vi "Orca Flash Data Spooler.vi"(7 "Calling VI Ref":refnum<vi>) -> ()   [LabVIEW 2016]
uses:
  <vilib>/vision/Image Controls.llb/IMAQ Image.ctl
  Orca Flash Capture Manager Controls/Orca Flash Capture Notifier Type.ctl
  Orca Flash Capture Manager Controls/Orca Flash Capture Actions.ctl
  Orca Flash Capture Manager Controls/Orca Flash Capture Switch Line Scan Modes.ctl
  Orca Flash Data Spooler/Orca Data Spooler Type Defs/Orca Data Spooler Notifier Type.ctl
  Orca Flash Data Spooler/Orca Data Spooler Type Defs/Orca Data Spooler Actions.ctl
  <vilib>/Utility/miscctls.llb/LVPointTypeDef.ctl
  Orca Flash Data Spooler/Orca Data Spooler Type Defs/Orca Data Spooler Transfer Data.ctl
  Orca Flash Data Spooler/Orca Data Spooler Type Defs/Orca Data Spooler Last Used.ctl
  Orca Flash Data Spooler/Orca Data Spooler Type Defs/Orca Data Spooler Transfer Log Type.ctl
  Tools/Copy File with Progress/Copy File DLL/x64/Release/Copy File DLL.dll
panel:
  in  "Main Tab":enum32{"Data Spooler", "Remote Queue"}(tab)
  out "Source Path":string
  out "Destination Path":string
  in  "Set Destination":bool
  in  "Disable Spooler":bool
  in  "Auto Match Paths":bool=TRUE
  in  "Skip File":bool
  in  "Abort":bool
  out "Copy Success":bool
  out "Current File":string
  out "Transfer Amount (%)":u8
  out "Spooler Active":bool
  out "Queue Started":bool
  in  "Open Queue":bool
  in  "Quit":bool
  out "Start Up Error":errorcluster
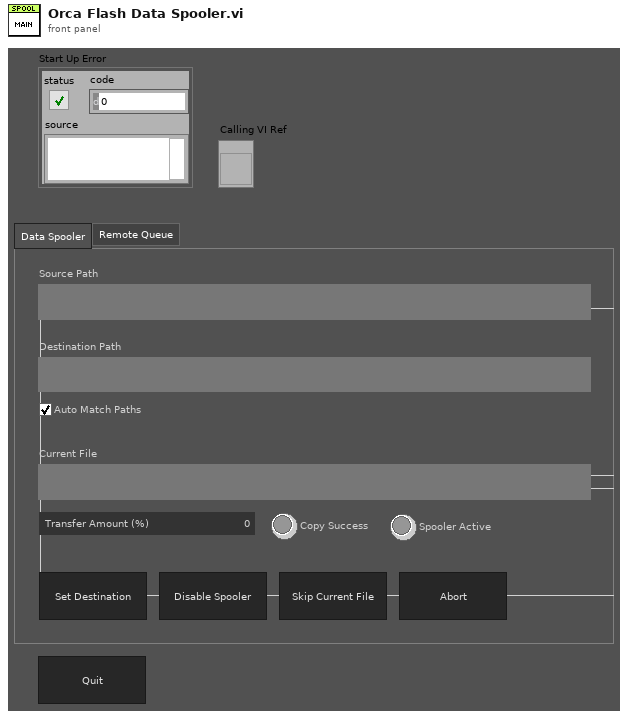
[diagram p1: front panel]
types:
  T1 = typedef "Orca Data Spooler Transfer Data.ctl" = cluster{"transLogPath":string, "imageName":string, "noFrames":u32, "noCycles":u16, "quitFlag":bool, "channelCode":u8, "setupName":string}
  T2 = enum16{"Always On", "Always Off", "Off While Running"}
  T3 = typedef "LVPointTypeDef.ctl" = cluster{"Horizontal":i16, "Vertical":i16}
  T4 = typedef "Orca Data Spooler Actions.ctl" = enum16{"Idle", "Start Spooler", "Update Destination", "Create Log File", "Wait for File", "Update Log", "Copy File", "Copy JSON Files", "Log Done", "Abort", "Exit", "Quit"}
  T5 = typedef "Orca Data Spooler Notifier Type.ctl" = cluster{"Actions":T4, "Source":path, "Destination":path, "Running?":bool, "Transfer Log":path}
  T6 = enum8{"Enabled", "Disabled", "Disabled and Grayed Out"}
  T7 = typedef "Orca Flash Capture Notifier Type.ctl" = cluster{"Actions":T8, "Running?":bool, "Preview Exposure (s)":dbl, "Capture Exposure (s)":dbl, "Cycles":u16, "Frames":u32, "No. of Z Steps":u16, "Z Step Size (µm)":dbl, "Base Path":path, "Init Z Position (µm)":dbl, "Lasers Lines":string[], "Save Path":path, "Line Scan?":bool, "Line Scan Mode":T9, "Collect Metadata?":bool, "channelCode":u8, "setupName":string}
  T8 = typedef "Orca Flash Capture Actions.ctl" = enum16{"Idle", "Live Preview", "Capture", "Check File Name", "Laser On", "Laser Off", "Open Shutters", "Close Shutters", "Set Exposure Time", "Start Acquisition", "Update SubFolder", "Write Metadata", "Setup", "Camera", "Switch", "Step", "Cycle", "External Cycle Sync", "Abort", "Quit"}
  T9 = typedef "Orca Flash Capture Switch Line Scan Modes.ctl" = enum32{"Automatic", "Use Presets", "Manual"}
  T10 = typedef "IMAQ Image.ctl" = refnum<image>
  T11 = cluster{"Image Ref":T10, "Cycle Number":u16, "Camera Running?":bool, "Capture?":bool}
  T12 = enum32{"Bad", "Idle", "Run top level", "Running"}
  T13 = typedef "Orca Data Spooler Last Used.ctl" = cluster{"Source":string, "Destination":string}
  T14 = typedef "LVRectTypeDef.ctl" = cluster{"Left":i16, "Top":i16, "Right":i16, "Bottom":i16}
  T15 = typedef "LVBoundsTypeDef.ctl" = cluster{"Width":u32, "Height":u32}
  T16 = enum16{"open", "replace", "create", "open or create", "replace or create", "replace or create with confirmation"}
  T17 = typedef "Orca Data Spooler Transfer Log Type.ctl" = cluster{"File Name":string, "Status":string}
  T18 = enum32{"Invalid", "Standard", "Closed", "Hidden", "Minimized", "Maximized"}
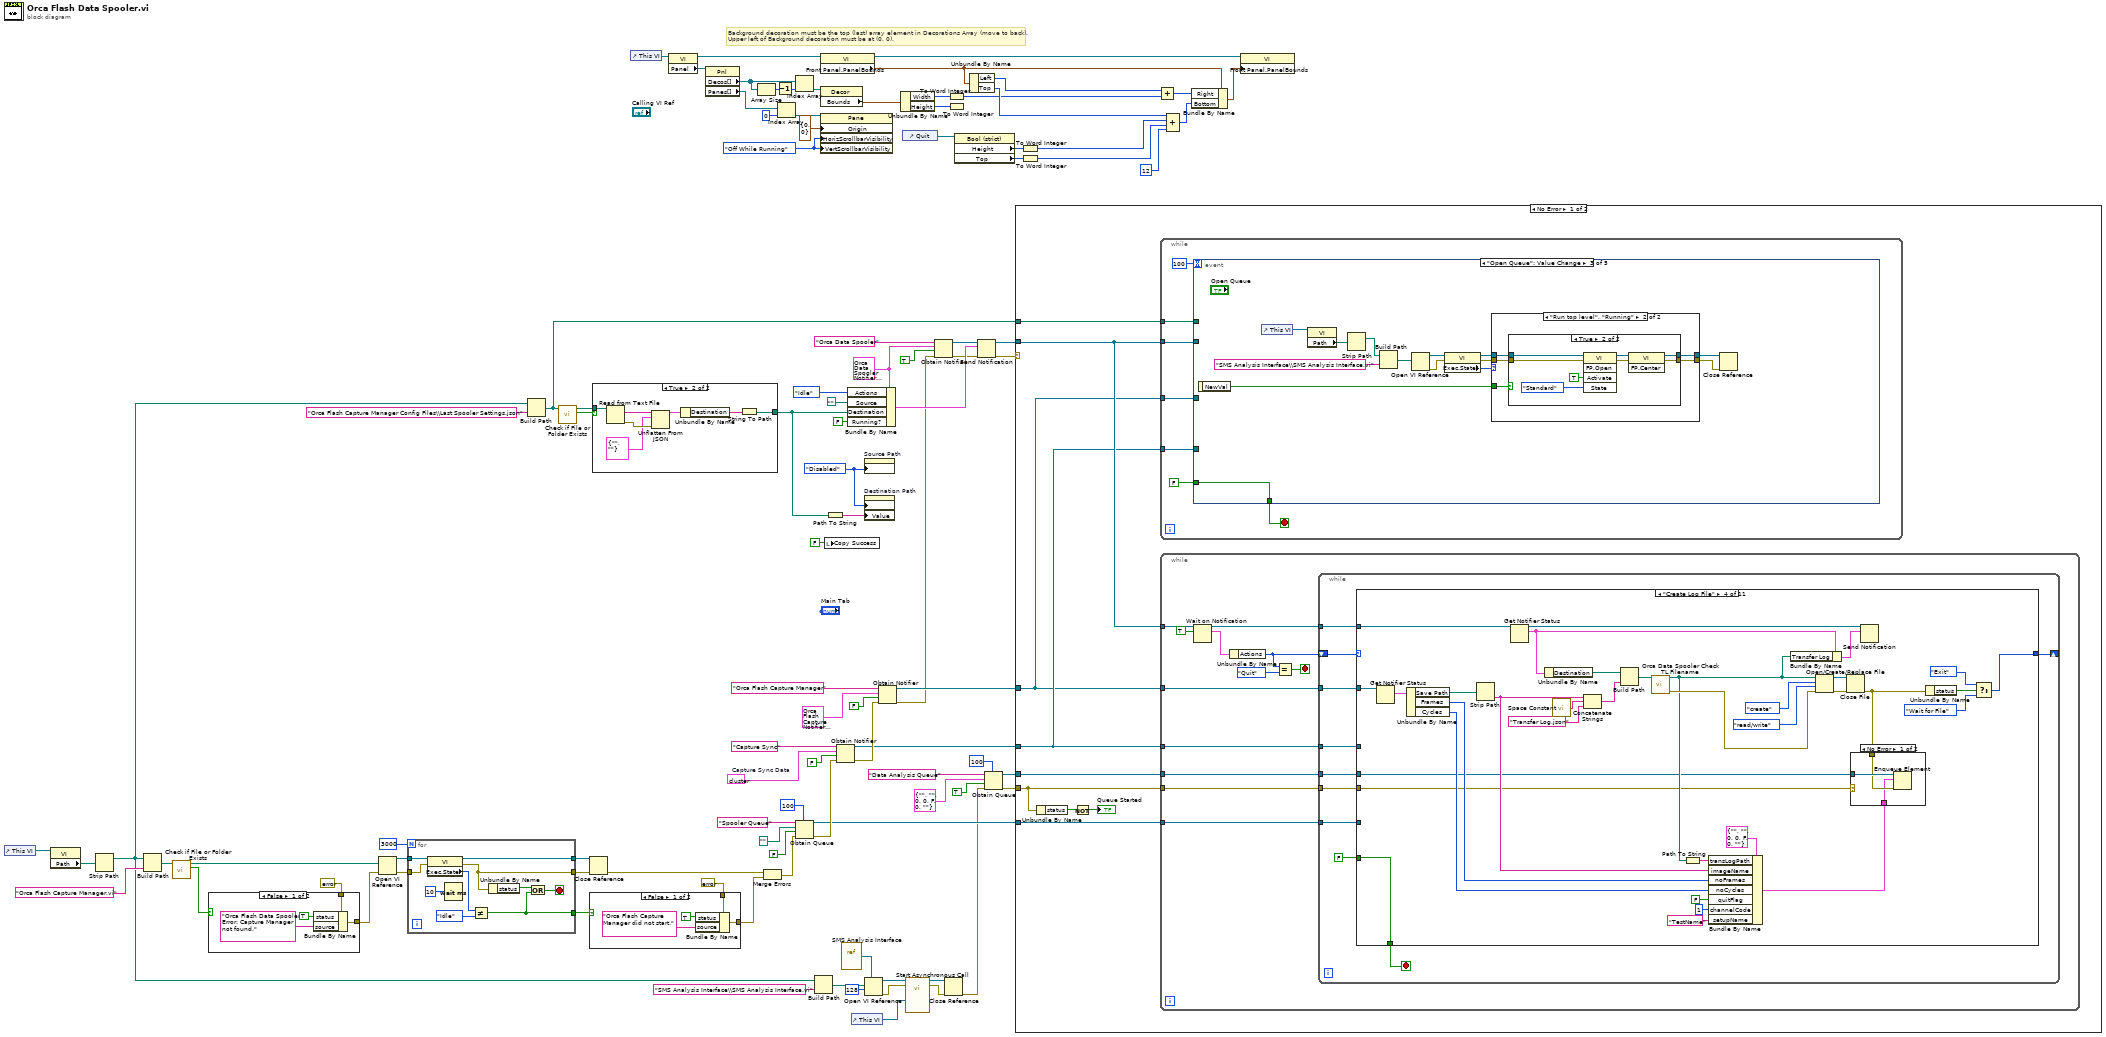
[diagram p0: block diagram]
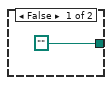
[diagram p2: hidden frame]
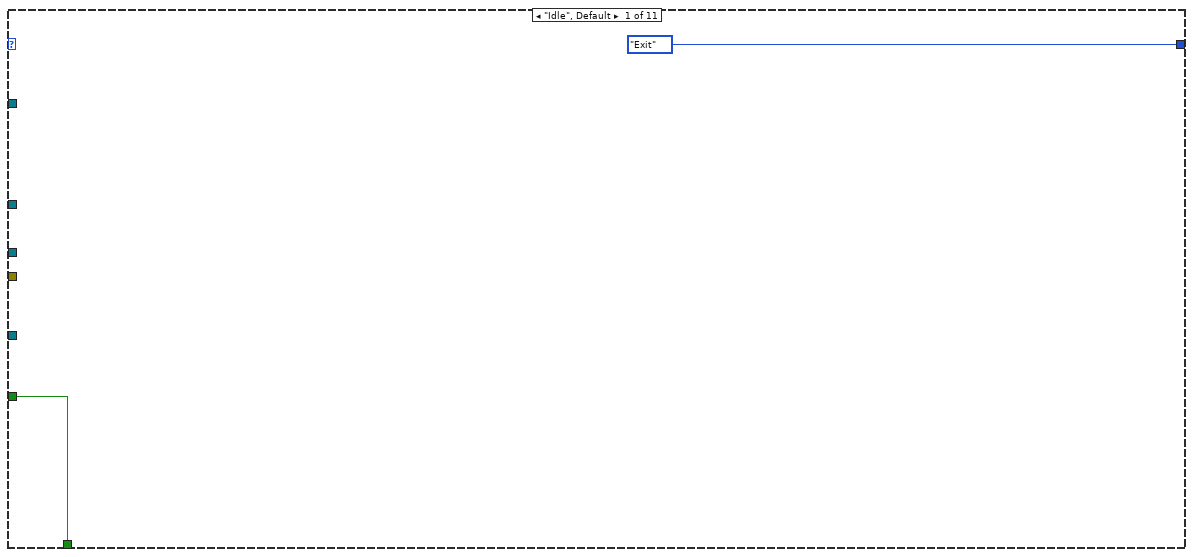
[diagram p3: hidden frame]
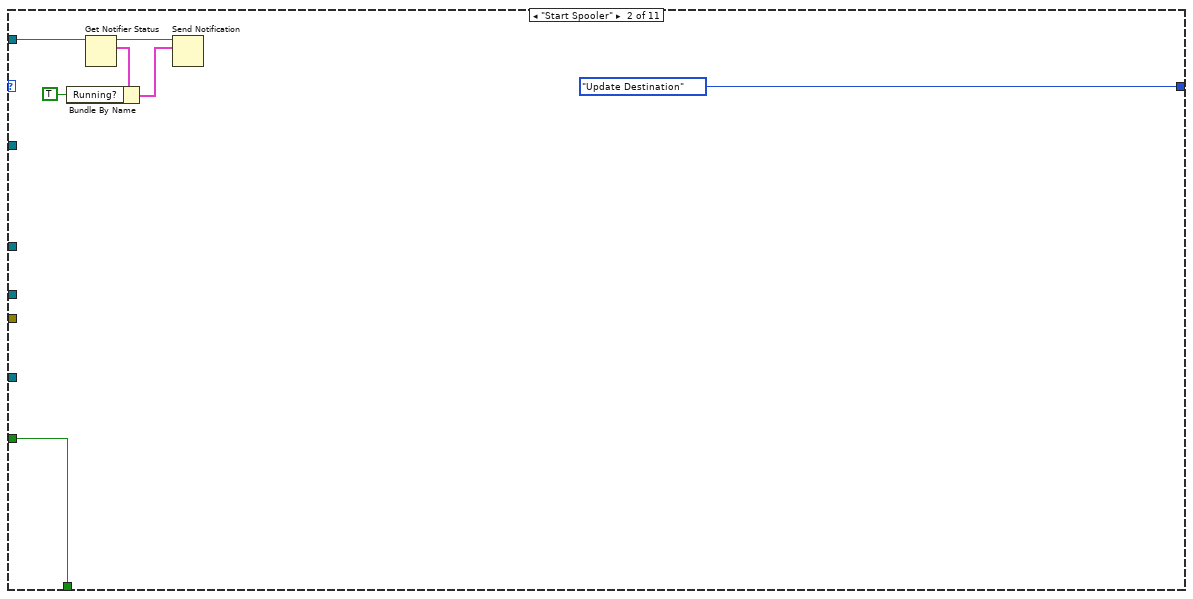
[diagram p4: hidden frame]
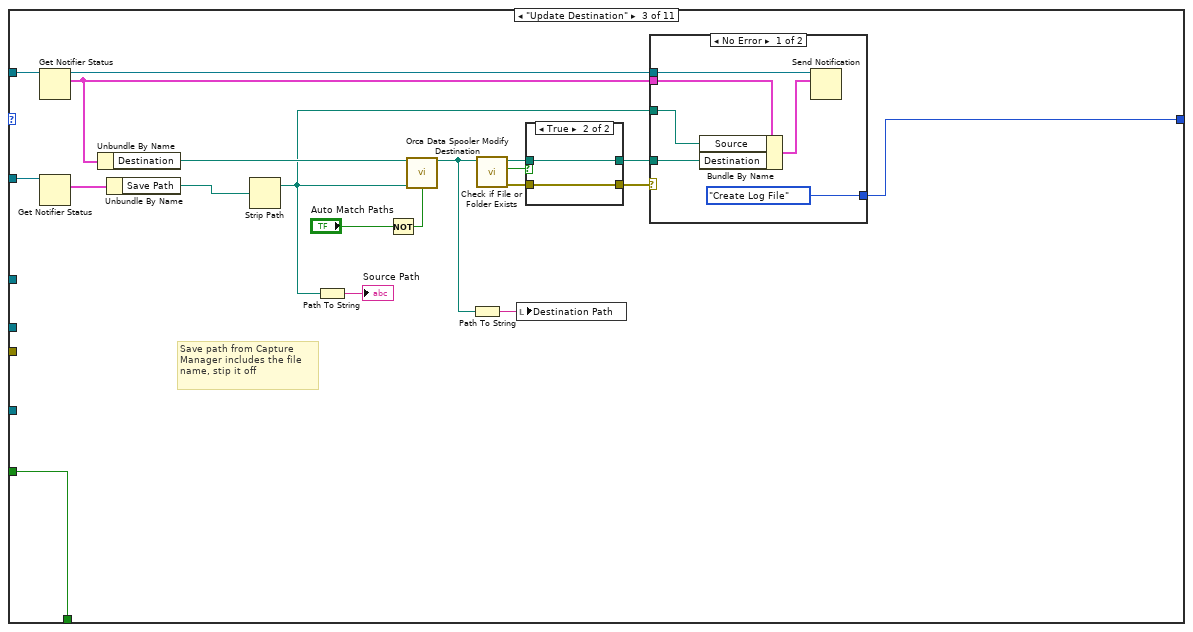
[diagram p5: hidden frame]
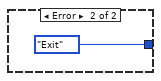
[diagram p6: hidden frame]
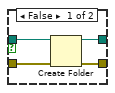
[diagram p7: hidden frame]
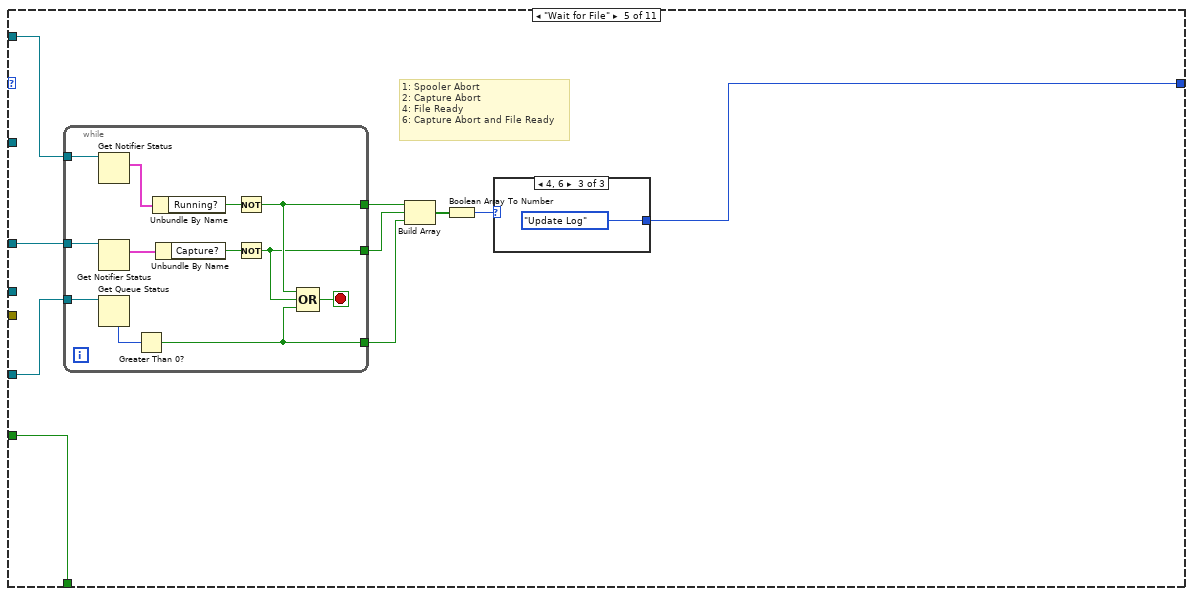
[diagram p9: hidden frame]
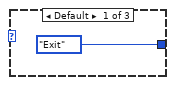
[diagram p10: hidden frame]
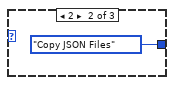
[diagram p11: hidden frame]
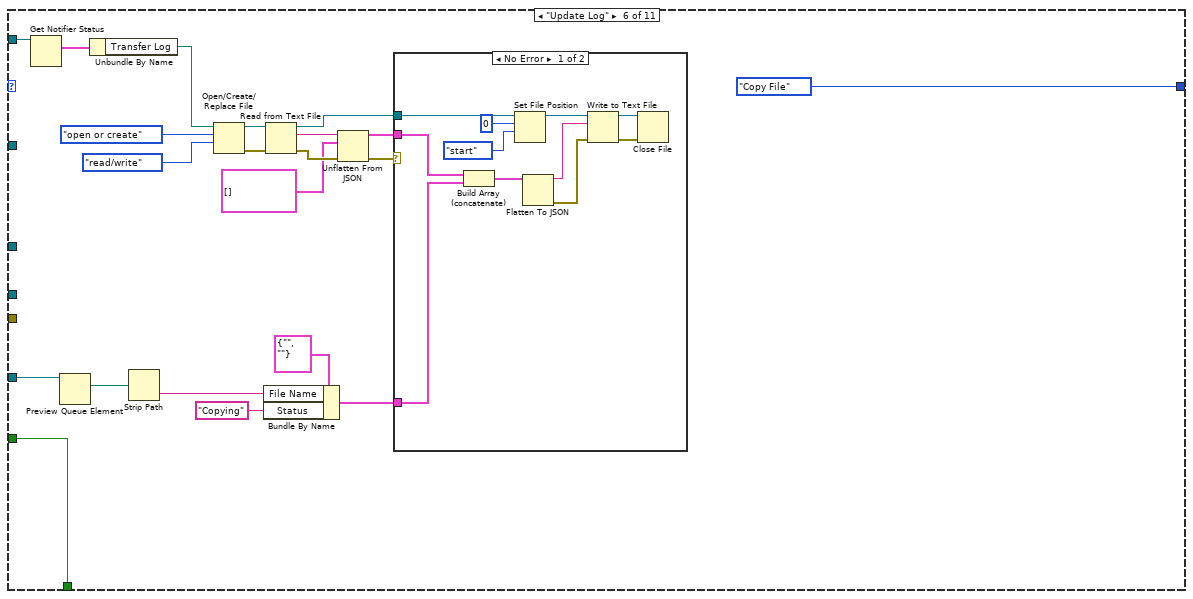
[diagram p12: hidden frame]
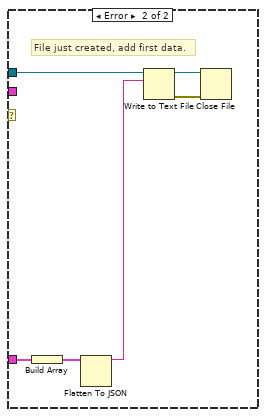
[diagram p13: hidden frame]
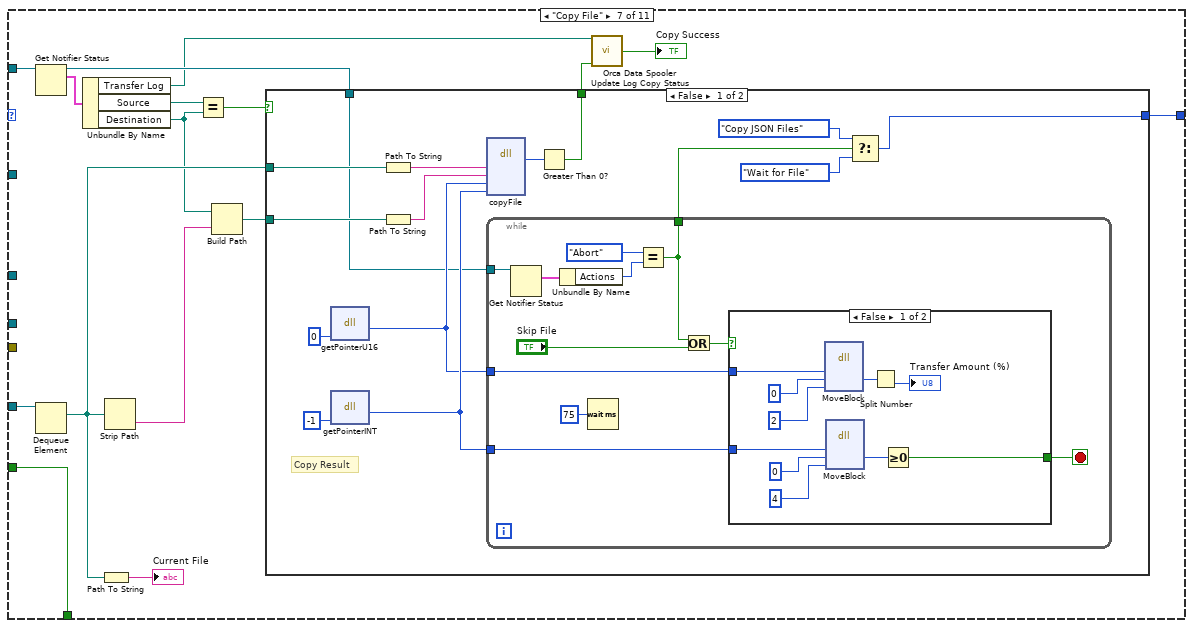
[diagram p14: hidden frame]
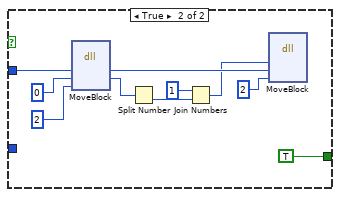
[diagram p15: hidden frame]
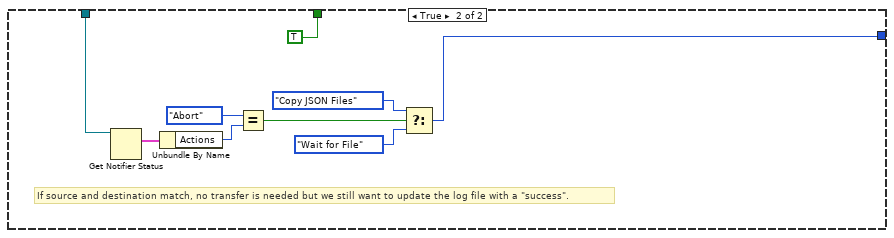
[diagram p16: hidden frame]
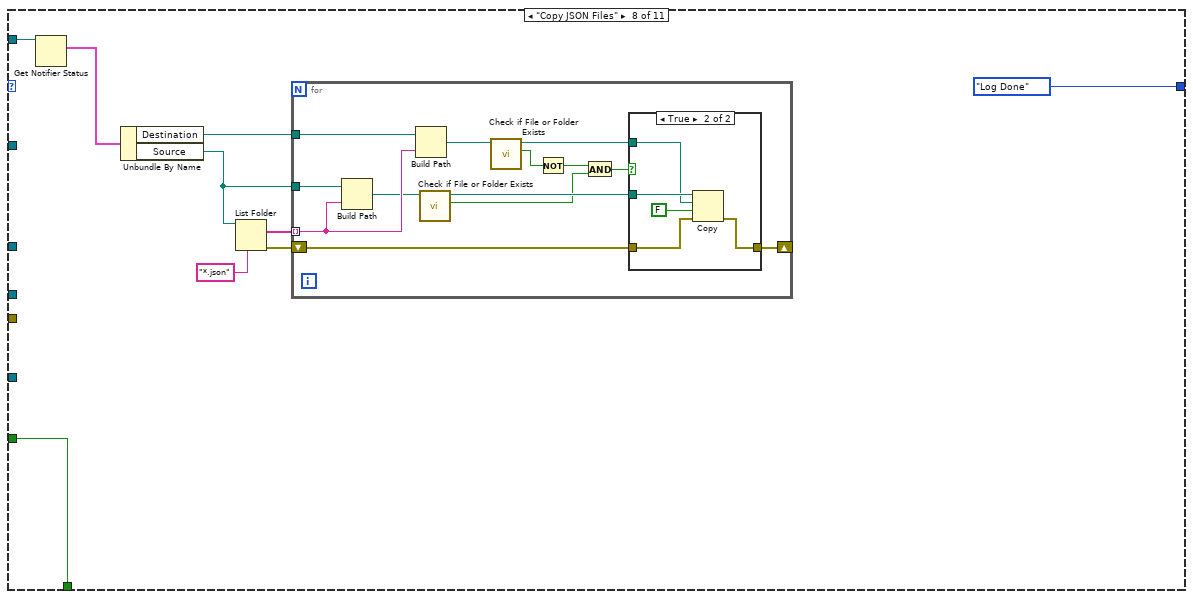
[diagram p17: hidden frame]
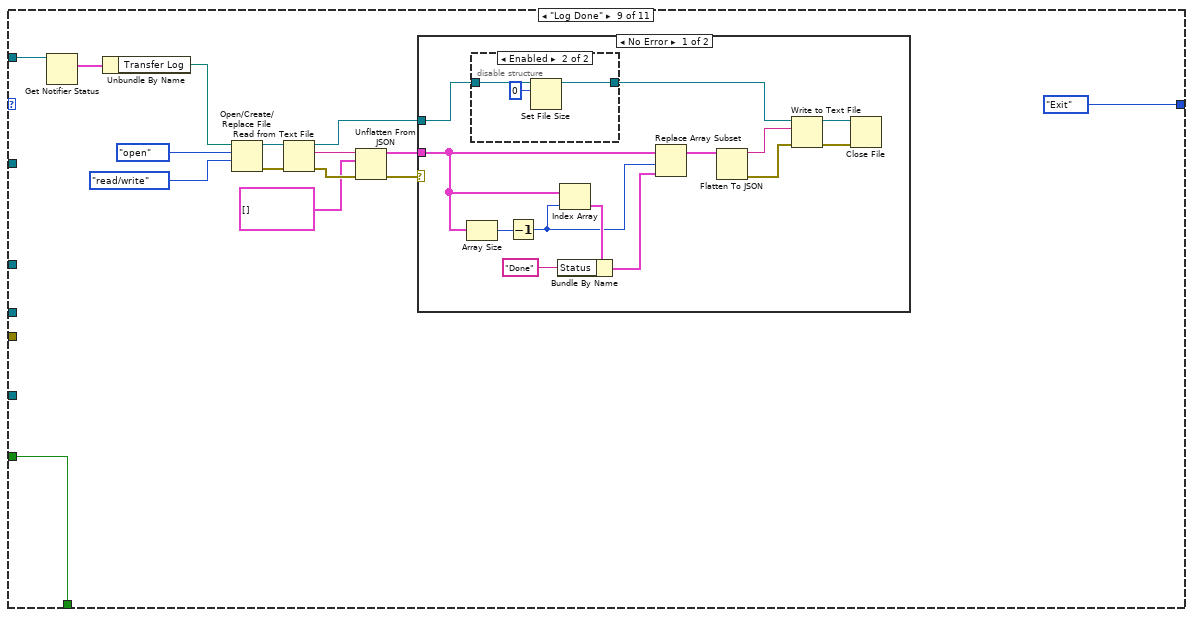
[diagram p19: hidden frame]
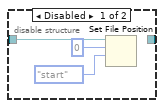
[diagram p20: hidden frame]
diagram:
  w39 = T2."Off While Running" ("Vertical Scrollbar Visibility")
  w65 = T5 {"Actions"=enum."Idle", "Source"=path "", "Destination"=path "", "Running?"=FALSE, "Transfer Log"=path ""} ("Orca Data Spooler Notifier Type")
  w71 = T6."Disabled" ("Disabled")
  w86 = T11 {"Image Ref"=refnum, "Cycle Number"=0, "Camera Running?"=FALSE, "Capture?"=FALSE}  # Capture Sync Data
  # "Background decoration must be the top (last) array element in Decorations Array (move to back).\nUpper left of Background decoration must be at (0, 0)."
  n1 = control-ref of="This VI"() -> (w99:refnum<vi>)
  n2 = property class="VI"(reference=w99) -> ("Path"=w98:path)  [unwired: 1 in, 2 out]
  n3 = Strip Path(path=w98) -> (stripped path=w10:path)  [unwired: 1 out]
  n4 = Build Path(base path=w10, name or relative path="Orca Flash Capture Manager.vi" ("name (unnamed)")) -> (appended path=w96:path)
  n5 = call <vilib>:"Check if File or Folder Exists.vi"("path"=w96) -> ("file or folder exists?"=w95:bool, "dup path"=w92:path)  [unwired: 8 in, 1 out]
  n6 = case shown="False" w95 {
    tunnel: errorcluster {"status"=FALSE, "code"=0, "source"=""} ("error in (no error)") -> [w101 w104]
    tunnel: [w100 w104] -> w91
    frame False {
      n7 = Bundle By Name(cluster=w101, "status"=TRUE, "source"="Orca Flash Data Spooler Error: Capture Manager not found." ("name (unnamed)")) -> (w100:errorcluster)
    }
    frame True {
    }
  }
  n8 = Open VI Reference(vi path=w92, error in (no error)=w91) -> (vi reference=w93:refnum<vi>, error out=w87:errorcluster)  [unwired: 4 in]
  n9 = for {
    N: 3000 -> [_]
    tunnel: w93 -> [w114]
    tunnel: [w110] -> w89
    tunnel: [w105] -> w79
    tunnel: [w107] -> w88
    tunnel: w87 -> [w106]
    stop <- w108 stop-if-true
    n10 = property class="VI"(reference=w114, error in=w106) -> (reference out=w110:refnum<vi>, error out=w107:errorcluster, "Exec.State"=w112:T12)
    n11 = Wait (ms)(milliseconds to wait=u32 10) -> ()  [unwired: 1 out]
    n12 = Not Equal?(x=w112, y=T12."Idle") -> (x != y?=w105:bool)
    n13 = Unbundle By Name(w107) -> ("status"=w109:bool)
    n14 = Or(x=w109, y=w105) -> (x .or. y?=w108:bool)
  }
  n15 = Build Path(base path=w10, name or relative path="Orca Flash Capture Manager Config Files\\Last Spooler Settings.json" ("name (unnamed)")) -> (appended path=w19:path)
  n16 = call <vilib>:"Check if File or Folder Exists.vi"("path"=w19) -> ("file or folder exists?"=w68:bool, "dup path"=w69:path)  [unwired: 8 in, 1 out]
  n17 = Close Reference(reference=w89, error in (no error)=w88) -> (error out=w78:errorcluster)
  n18 = case shown="False" w79 {
    tunnel: errorcluster {"status"=FALSE, "code"=0, "source"=""} ("error in (no error)") -> [w116 w119]
    tunnel: [w115 w119] -> w77
    frame False {
      n19 = Bundle By Name(cluster=w116, "status"=TRUE, "source"="Orca Flash Capture Manager did not start." ("name (unnamed)")) -> (w115:errorcluster)
    }
    frame True {
    }
  }
  n20 = case shown="True" w68 {
    tunnel: w69 -> [_ w125]
    tunnel: [path "" w121] -> w61
    frame False {
    }
    frame True {
      n21 = Read from Text File(file (use dialog)=w125) -> (text=w127:string, error out=w126:errorcluster)  [unwired: 3 in, 2 out]
      n22 = Unflatten From JSON(JSON string=w127, type and defaults=T13 {"Source"="", "Destination"=""} ("Orca Data Spooler Notifier Type"), error in (no error)=w126) -> (value=w123:T13)  [unwired: 4 in, 1 out]
      n23 = Unbundle By Name(w123) -> ("Destination"=w122:string)
      n24 = String To Path(string=w122) -> (path=w121:path)
    }
  }
  n25 = control-ref of="This VI"() -> (w31:refnum<vi>)
  n26 = property class="VI"(reference=w31) -> (reference out=w40:refnum<vi>, "Panel"=w32:refnum<vi>)  [unwired: 1 in, 1 out]
  n27 = property class="Pnl"(reference=w32) -> ("Decos[]"=w30:refnum<vi>[], "Panes[]"=w36:refnum<vi>[])  [unwired: 1 in, 2 out]
  n28 = Array Size(array=w30) -> (size(s)=w28:i32)
  n29 = Merge Errors(w78, w77) -> (w22:errorcluster)
  n30 = Decrement(x=w28) -> (x-1=w29:i32)
  n31 = Index Array(array=w36, index=0) -> (element=w35:refnum<vi>)
  n32 = Index Array(array=w30, index=w29) -> (element=w38:refnum<vi>)
  n33 = Obtain Queue(max queue size (-1, unlimited)=100, name (unnamed)="Spooler Queue", element data type=path "", create if not found? (T)=FALSE, error in (no error)=w22) -> (queue out=w20:refnum<queue>, error out=w21:errorcluster)  [unwired: 1 out]
  n34 = Build Path(base path=w10, name or relative path="SMS Analysis Interface\\SMS Analysis Interface.vi" ("name (unnamed)")) -> (appended path=w11:path)
  n35 = property class="VI"(reference=w40) -> (reference out=w42:refnum<vi>, "Front Panel.PanelBounds"=w43:T14)  [unwired: 1 in, 1 out]
  n36 = property class="Decor"(reference=w38) -> ("Bounds"=w41:T15)  [unwired: 1 in, 2 out]
  n37 = property class="Pane"(reference=w35, "Origin"=T3 {"Horizontal"=0, "Vertical"=0}, "HorizScrollbarVisibility"=w39, "VertScrollbarVisibility"=w39) -> ()  [unwired: 1 in, 2 out]
  n38 = local write "Copy Success"(FALSE ("Copy Success")) -> ()
  n39 = Path To String(path=w61) -> (string=w60:string)
  n40 = Obtain Notifier(name (unnamed)="Capture Sync", notification data type=w86, create if not found? (T)=FALSE, error in (no error)=w21) -> (notifier out=w74:refnum<notifier>, error out=w76:errorcluster)  [unwired: 1 out]
  n41 = vi-ref "SMS Analysis Interface.vi"() -> (w9:refnum<vi>)
  n42 = Bundle By Name(cluster=w65, "Actions"=Orca_Data_Spooler_Actions."Idle", "Source"=path "", "Destination"=w61, "Running?"=FALSE) -> (w63:T5)
  n43 = control-ref of="This VI"() -> (w3:refnum<vi>)
  n44 = property on="Source Path" class="Str"("DisabledEnum"=w71) -> ()  [unwired: 2 in, 2 out]
  n45 = property on="Destination Path" class="Str"("DisabledEnum"=w71, "Value"=w60) -> ()  [unwired: 2 in, 2 out]
  n46 = Open VI Reference(type specifier VI Refnum (for type only)=w9, vi path=w11, options=128) -> (vi reference=w7:refnum<vi>, error out=w5:errorcluster)  [unwired: 3 in]
  n47 = Obtain Notifier(name (unnamed)="Orca Flash Capture Manager", notification data type=T7 {"Actions"=enum."Live Preview", "Running?"=FALSE, "Preview Exposure (s)"=0.1, "Capture Exposure (s)"=0.1, "Cycles"=1, "Frames"=0, "No. of Z Steps"=0, "Z Step Size (µm)"=0.0, "Base Path"=path "", "Init Z Position (µm)"=0.0, "Lasers Lines"=[], "Save Path"=path "", "Line Scan?"=FALSE, "Line Scan Mode"=enum."Automatic", "Collect Metadata?"=FALSE, "channelCode"=0, "setupName"=""} ("4Pi Capture Notifier Type"), create if not found? (T)=FALSE, error in (no error)=w76) -> (notifier out=w75:refnum<notifier>, error out=w59:errorcluster)  [unwired: 1 out]
  n48 = Unbundle By Name(w41) -> ("Width"=w46:u32, "Height"=w49:u32)
  n49 = control-ref of="Quit"() -> (w33:refnum<vi>)
  n50 = call-by-ref "Start Asynchronous Call"(reference=w7, error in=w5, "Calling VI Ref"=w3) -> (reference out=w6:refnum<vi>, error out=w4:errorcluster)  [unwired: 15 in]
  n51 = Obtain Notifier(name (unnamed)="Orca Data Spooler", notification data type=w65, create if not found? (T)=TRUE, error in (no error)=w59) -> (notifier out=w64:refnum<notifier>, error out=w62:errorcluster)  [unwired: 1 out]
  n52 = Close Reference(reference=w6, error in (no error)=w4) -> (error out=w2:errorcluster)
  n53 = To Word Integer(number=w46) -> (16bit integer=w48:i16)
  n54 = To Word Integer(number=w49) -> ()  [unwired: 1 out]
  n55 = property class="Bool (strict)"(reference=w33) -> ("Height"=w51:u32, "Top"=w52:i32)  [unwired: 1 in, 2 out]
  n56 = Unbundle By Name(w43) -> ("Left"=w45:i16, "Top"=w56:i16)
  n57 = Send Notification(notification=w63, notifier=w64, error in (no error)=w62) -> (notifier out=w57:refnum<notifier>, error out=w58:errorcluster)
  n58 = Obtain Queue(max queue size (-1, unlimited)=100, name (unnamed)="Data Analysis Queue", element data type=T1 {"transLogPath"="", "imageName"="", "noFrames"=0, "noCycles"=0, "quitFlag"=FALSE, "channelCode"=0, "setupName"=""} ("Spooler Connection Data"), create if not found? (T)=TRUE, error in (no error)=w2) -> (queue out=w13:refnum<queue>, error out=w1:errorcluster)  [unwired: 1 out]
  n59 = case shown="No Error" w58 {
    selector: w58 -> [_ w552]
    tunnel: w75 -> [w134 w550]
    tunnel: w74 -> [w135 w548]
    tunnel: w57 -> [w136 w549]
    tunnel: w20 -> [w133 _]
    tunnel: w19 -> [w132 _]
    tunnel: w13 -> [w131 _]
    tunnel: w1 -> [w130 _]
    frame No Error {
      n60 = Unbundle By Name(w130) -> ("status"=w129:bool)
      n61 = Not(x=w129) -> (.not. x?=→"Queue Started":bool)
      n62 = while {
        tunnel: w136 -> [w452]
        tunnel: w134 -> [w451]
        tunnel: w135 -> [w450]
        tunnel: w132 -> [w448]
        stop <- w453 stop-if-true
        n63 = event shown="[2] \"Open Queue\": Value Change" {
          selector: _ -> [_ _ _ _ _]
          dyn-events: _ -> [_ _ _ _ _]
          timeout: 100 -> [_ _ _ _ _]
          tunnel: FALSE -> [w473 w488 w514 w539 _]
          tunnel: [w473 w488 w514 w539 w545] -> w453
          tunnel: w452 -> [w462 w487 _ w535 w544]
          tunnel: w451 -> [w472 _ _ _ _]
          tunnel: w450 -> [w471 _ _ _ _]
          tunnel: w448 -> [_ w481 _ _ _]
          event Timeout {
            n64 = event-data() -> ()  [unwired: 1 in, 1 out]
            n65 = Get Notifier Status(notifier=w462) -> (notifier out=w459:refnum<notifier>, current notification=w461:T5)  [unwired: 1 in, 3 out]
            n66 = Get Notifier Status(notifier=w472) -> (current notification=w470:T7)  [unwired: 1 in, 4 out]
            n67 = Get Notifier Status(notifier=w471) -> (current notification=w467:T11)  [unwired: 1 in, 4 out]
            n68 = Unbundle By Name(w467) -> ("Capture?"=w464:bool, "Camera Running?"=w465:bool)
            n69 = Unbundle By Name(w461) -> ("Running?"=w455:bool)
            "Spooler Active" <- w455
            n70 = Unbundle By Name(w470) -> ("Actions"=w469:T8, "Base Path"=w456:path)
            n71 = case shown="False" w455 {
              tunnel: w456 -> [w474 _]
              frame False {
                n72 = Path To String(path=w474) -> (string=w475:string)
                n73 = local write "Source Path"(w475) -> ()
              }
              frame True {
              }
            }
            n74 = Not(x=w455) -> (.not. x?=w460:bool)
            n75 = Equal?(x=Orca_Flash_Capture_Actions."Capture", y=w469) -> (x = y?=w466:bool)
            n76 = Not(x="Disable Spooler") -> (.not. x?=w457:bool)
            n77 = Compound Arithmetic op=AND(w460, w466, w464, w465, w457) -> (w463:bool)
            n78 = case shown="True" w463 {
              tunnel: w459 -> [_ w480]
              frame False {
              }
              frame True {
                n79 = Get Notifier Status(notifier=w480) -> (notifier out=w479:refnum<notifier>, current notification=w478:T5)  [unwired: 1 in, 3 out]
                n80 = Bundle By Name(cluster=w478, "Actions"=Orca_Data_Spooler_Actions."Start Spooler") -> (w477:T5)
                n81 = Send Notification(notification=w477, notifier=w479) -> ()  [unwired: 1 in, 2 out]
              }
            }
          }
          event "Set Destination": Value Change {
            n82 = event-data() -> ()  [unwired: 1 in, 1 out]
            n83 = Get Notifier Status(notifier=w487) -> (notifier out=w483:refnum<notifier>, current notification=w486:T5)  [unwired: 1 in, 3 out]
            n84 = Unbundle By Name(w486) -> ("Destination"=w485:path)
            n85 = call "File Dialog"("start path"=w485) -> ("selected path"=w482:path, "error out"=w484:errorcluster)  [unwired: 11 in, 2 out]
            n86 = case shown="No Error" w484 {
              tunnel: w483 -> [w500 _]
              tunnel: w482 -> [w498 _]
              tunnel: w481 -> [w496 _]
              frame No Error {
                n87 = Path To String(path=w498) -> (string=w493:string)
                "Destination Path" <- w493
                n88 = Get Notifier Status(notifier=w500) -> (notifier out=w497:refnum<notifier>, current notification=w499:T5)  [unwired: 1 in, 3 out]
                n89 = Bundle By Name(cluster=w499, "Destination"=w498) -> (w492:T5)
                n90 = Send Notification(notification=w492, notifier=w497) -> ()  [unwired: 1 in, 2 out]
                n91 = Unbundle By Name(w492) -> ("Source"=w490:path)
                n92 = Path To String(path=w490) -> (string=w491:string)
                n93 = Bundle By Name(cluster=T13 {"Source"="", "Destination"=""} ("Orca Data Spooler Notifier Type"), "Source"=w491, "Destination"=w493) -> (w495:T13)
                n94 = Flatten To JSON(anything=w495) -> (JSON string=w489:string)  [unwired: 2 in, 1 out]
                n95 = Write to Text File(file (use dialog)=w496, text=w489) -> ()  [unwired: 2 in, 3 out]
              }
              frame Error {
              }
            }
          }
          event "Open Queue": Value Change {
            n96 = event-data() -> ("NewVal"=w504:bool)  [unwired: 1 in]
            n97 = control-ref of="This VI"() -> (w513:refnum<vi>)
            n98 = property class="VI"(reference=w513) -> ("Path"=w512:path)  [unwired: 1 in, 2 out]
            n99 = Strip Path(path=w512) -> (stripped path=w510:path)  [unwired: 1 out]
            n100 = Build Path(base path=w510, name or relative path="SMS Analysis Interface\\SMS Analysis Interface.vi" ("name (unnamed)")) -> (appended path=w509:path)
            n101 = Open VI Reference(vi path=w509) -> (vi reference=w508:refnum<vi>, error out=w507:errorcluster)  [unwired: 5 in]
            n102 = property class="VI"(reference=w508, error in=w507) -> (reference out=w506:refnum<vi>, error out=w503:errorcluster, "Exec.State"=w505:T12)
            n103 = case shown="\"Run top level\", \"Running\"" w505 {
              tunnel: w506 -> [w516 w520]
              tunnel: w503 -> [w515 w521]
              tunnel: [w516 w519] -> w502
              tunnel: [w515 w518] -> w501
              tunnel: w504 -> [_ w517]
              frame Default {
              }
              frame "Run top level", "Running" {
                n104 = case shown="True" w517 {
                  tunnel: w521 -> [w523 w532]
                  tunnel: w520 -> [w525 w531]
                  tunnel: [w524 w527] -> w519
                  tunnel: [w522 w526] -> w518
                  frame False {
                    n105 = invoke class="VI" method="FP.Close"(reference=w525, error in=w523) -> (reference out=w524:refnum<vi>, error out=w522:errorcluster)  [unwired: 1 in, 1 out]
                  }
                  frame True {
                    n106 = invoke class="VI" method="FP.Open"(reference=w531, error in=w532, "Activate"=TRUE ("Activate?"), "State"=T18."Standard") -> (reference out=w529:refnum<vi>, error out=w528:errorcluster)  [unwired: 1 in, 3 out]
                    n107 = invoke class="VI" method="FP.Center"(reference=w529, error in=w528) -> (reference out=w527:refnum<vi>, error out=w526:errorcluster)  [unwired: 1 in, 1 out]
                  }
                }
              }
            }
            n108 = Close Reference(reference=w502, error in (no error)=w501) -> ()  [unwired: 1 out]
          }
          event "Abort": Value Change {
            n109 = event-data() -> ()  [unwired: 1 in, 1 out]
            n110 = Get Notifier Status(notifier=w535) -> (notifier out=w538:refnum<notifier>, current notification=w537:T5)  [unwired: 1 in, 3 out]
            n111 = Bundle By Name(cluster=w537, "Actions"=Orca_Data_Spooler_Actions."Abort") -> (w536:T5)
            n112 = Send Notification(notification=w536, notifier=w538) -> ()  [unwired: 1 in, 2 out]
          }
          event "Quit": Value Change {
            n113 = event-data() -> ("NewVal"=w545:bool)  [unwired: 1 in]
            n114 = Get Notifier Status(notifier=w544) -> (notifier out=w542:refnum<notifier>, current notification=w543:T5)  [unwired: 1 in, 3 out]
            n115 = Bundle By Name(cluster=w543, "Actions"=Orca_Data_Spooler_Actions."Quit") -> (w541:T5)
            n116 = Send Notification(notification=w541, notifier=w542) -> ()  [unwired: 1 in, 2 out]
          }
        }
      }
      n117 = while {
        tunnel: w136 -> [w148]
        tunnel: w135 -> [w141]
        tunnel: w134 -> [w140]
        tunnel: w133 -> [w139]
        tunnel: w131 -> [w138]
        tunnel: w130 -> [w137]
        stop <- w144 stop-if-true
        n118 = Wait on Notification(notifier=w148, ignore previous (F)=TRUE) -> (notifier out=w142:refnum<notifier>, notification=w146:T5)  [unwired: 2 in, 2 out]
        n119 = Unbundle By Name(w146) -> ("Actions"=w143:T4)
        n120 = Equal?(x=w143, y=Orca_Data_Spooler_Actions."Quit") -> (x = y?=w144:bool)
        n121 = while {
          shift-right: [w154] -> _
          shift-left: w143 -> [w158]
          tunnel: w142 -> [w157]
          tunnel: w141 -> [w153]
          tunnel: w140 -> [w152]
          tunnel: w139 -> [w151]
          tunnel: w138 -> [w150]
          tunnel: w137 -> [w149]
          stop <- w155 stop-if-true
          n122 = case shown="\"Create Log File\"" w158 {
            tunnel: w157 -> [_ w165 w184 w228 w246 w281 w315 w380 w401 w436 w443]
            tunnel: FALSE -> [w160 w167 w187 w229 w248 w284 w317 w381 w415 w442 w447]
            tunnel: [w160 w167 w187 w229 w248 w284 w317 w381 w415 w441 w446] -> w155
            tunnel: [Orca_Data_Spooler_Actions."Exit" ("y") Orca_Data_Spooler_Actions."Update Destination" ("y") w171 w222 w239 Orca_Data_Spooler_Actions."Copy File" ("y") w308 Orca_Data_Spooler_Actions."Log Done" ("y") Orca_Data_Spooler_Actions."Exit" ("y") Orca_Data_Spooler_Actions."Exit" ("y") Orca_Data_Spooler_Actions."Quit" ("y")] -> w154
            tunnel: w153 -> [_ _ _ _ w245 _ _ _ _ _ _]
            tunnel: w152 -> [_ _ w186 w216 _ _ _ _ _ _ _]
            tunnel: w151 -> [_ _ _ _ w247 w282 w316 _ _ _ _]
            tunnel: w150 -> [_ _ _ w206 _ _ _ _ _ _ w444]
            tunnel: w149 -> [_ _ _ w203 _ _ _ _ _ _ _]
            frame "Idle", Default {
            }
            frame "Start Spooler" {
              n123 = Get Notifier Status(notifier=w165) -> (notifier out=w163:refnum<notifier>, current notification=w164:T5)  [unwired: 1 in, 3 out]
              n124 = Bundle By Name(cluster=w164, "Running?"=TRUE) -> (w161:T5)
              n125 = Send Notification(notification=w161, notifier=w163) -> ()  [unwired: 1 in, 2 out]
            }
            frame "Update Destination" {
              # "Save path from Capture Manager includes the file name, stip it off"
              n126 = Get Notifier Status(notifier=w184) -> (notifier out=w182:refnum<notifier>, current notification=w181:T5)  [unwired: 1 in, 3 out]
              n127 = Get Notifier Status(notifier=w186) -> (current notification=w185:T7)  [unwired: 1 in, 4 out]
              n128 = Unbundle By Name(w181) -> ("Destination"=w179:path)
              n129 = Unbundle By Name(w185) -> ("Save Path"=w169:path)
              n130 = Strip Path(path=w169) -> (stripped path=w168:path)  [unwired: 1 out]
              n131 = Path To String(path=w168) -> (string=→"Source Path":string)
              n132 = Not(x="Auto Match Paths") -> (.not. x?=w170:bool)
              n133 = call "Orca Data Spooler Modify Destination.vi"("Destination"=w179, "Source"=w168, "Ignore Source?"=w170) -> ("Modified Destination"=w177:path)  [unwired: 12 in]
              n134 = Path To String(path=w177) -> (string=w180:string)
              n135 = call <vilib>:"Check if File or Folder Exists.vi"("path"=w177) -> ("error out"=w174:errorcluster, "file or folder exists?"=w176:bool, "dup path"=w175:path)  [unwired: 8 in]
              n136 = local write "Destination Path"(w180) -> ()
              n137 = case shown="True" w176 {
                tunnel: w175 -> [w198 w199]
                tunnel: w174 -> [w197 w200]
                tunnel: [w196 w200] -> w173
                tunnel: [w195 w199] -> w172
                frame False {
                  n138 = Create Folder(path (use dialog)=w198, error in=w197) -> (created path=w195:path, error out=w196:errorcluster)  [unwired: 1 in, 1 out]
                }
                frame True {
                }
              }
              n139 = case shown="No Error" w173 {
                tunnel: w182 -> [w193 _]
                tunnel: w181 -> [w192 _]
                tunnel: w172 -> [w190 _]
                tunnel: [Orca_Data_Spooler_Actions."Create Log File" ("y") Orca_Data_Spooler_Actions."Exit" ("y")] -> w171
                tunnel: w168 -> [w188 _]
                frame No Error {
                  n140 = Bundle By Name(cluster=w192, "Source"=w188, "Destination"=w190) -> (w191:T5)
                  n141 = Send Notification(notification=w191, notifier=w193) -> ()  [unwired: 1 in, 2 out]
                }
                frame Error {
                }
              }
            }
            frame "Create Log File" {
              n142 = Get Notifier Status(notifier=w216) -> (current notification=w218:T7)  [unwired: 1 in, 4 out]
              n143 = Unbundle By Name(w218) -> ("Save Path"=w217:path, "Frames"=w207:u32, "Cycles"=w208:u16)
              n144 = Strip Path(path=w217) -> (name=w211:string)  [unwired: 1 out]
              n145 = Get Notifier Status(notifier=w228) -> (notifier out=w231:refnum<notifier>, current notification=w232:T5)  [unwired: 1 in, 3 out]
              n146 = Unbundle By Name(w232) -> ("Destination"=w235:path)
              n147 = call <vilib>:"Space Constant.vi"() -> ("String"=w220:string)
              n148 = Concatenate Strings(w211, w220, "Transfer Log.json" ("name or relative path")) -> (w219:string)
              n149 = Build Path(base path=w235, name or relative path=w219) -> (appended path=w215:path)
              n150 = call "Orca Data Spooler Check TL Filename.vi"("Path"=w215) -> ("Proof Path"=w209:path, "Error Out"=w214:errorcluster)  [unwired: 13 in]
              n151 = Path To String(path=w209) -> (string=w210:string)
              n152 = Bundle By Name(cluster=T1 {"transLogPath"="", "imageName"="", "noFrames"=0, "noCycles"=0, "quitFlag"=FALSE, "channelCode"=0, "setupName"=""} ("Spooler Connection Data"), "transLogPath"=w210, "imageName"=w211, "noFrames"=w207, "noCycles"=w208, "quitFlag"=FALSE, "channelCode"=u8 1, "setupName"="TestName") -> (w204:T1)
              n153 = Bundle By Name(cluster=w232, "Transfer Log"=w209) -> (w230:T5)
              n154 = Open/Create/Replace File(file path (use dialog)=w209, error in=w214, operation (0:open)=T16."create", access (0:read/write)=enum16{"read/write", "read-only", "write-only"}."read/write") -> (refnum out=w227:refnum<file>, error out=w226:errorcluster)  [unwired: 2 in, 1 out]
              n155 = Close File(refnum=w227, error in=w226) -> (error out=w205:errorcluster)  [unwired: 1 out]
              n156 = case shown="No Error" w203 {
                tunnel: w206 -> [w238 _]
                tunnel: w205 -> [w237 _]
                tunnel: w204 -> [w236 _]
                frame No Error {
                  n157 = Enqueue Element(queue=w238, element=w236, error in (no error)=w237) -> ()  [unwired: 1 in, 3 out]
                }
                frame Error {
                }
              }
              n158 = Send Notification(notification=w230, notifier=w231) -> ()  [unwired: 1 in, 2 out]
              n159 = Unbundle By Name(w205) -> ("status"=w225:bool)
              n160 = Select(t=Orca_Data_Spooler_Actions."Exit" ("y"), s=w225, f=Orca_Data_Spooler_Actions."Wait for File" ("y")) -> (s? t:f=w222:T4)
            }
            frame "Wait for File" {
              # "1: Spooler Abort\n2: Capture Abort\n4: File Ready\n6: Capture Abort and File Ready"
              n161 = while {
                tunnel: w247 -> [w262]
                tunnel: w246 -> [w263]
                tunnel: [w253] -> w244
                tunnel: w245 -> [w259]
                tunnel: [w252] -> w242
                tunnel: [w256] -> w243
                stop <- w257 stop-if-true
                n162 = Get Notifier Status(notifier=w263) -> (current notification=w260:T5)  [unwired: 1 in, 4 out]
                n163 = Get Notifier Status(notifier=w259) -> (current notification=w258:T11)  [unwired: 1 in, 4 out]
                n164 = Get Queue Status(queue=w262) -> (# elements in queue=w261:i32)  [unwired: 2 in, 7 out]
                n165 = Greater Than 0?(x=w261) -> (x > 0?=w256:bool)
                n166 = Unbundle By Name(w260) -> ("Running?"=w254:bool)
                n167 = Unbundle By Name(w258) -> ("Capture?"=w255:bool)
                n168 = Not(x=w254) -> (.not. x?=w253:bool)
                n169 = Not(x=w255) -> (.not. x?=w252:bool)
                n170 = Compound Arithmetic op=OR(w253, w252, w256) -> (w257:bool)
              }
              n171 = Build Array(w244, w242, w243) -> (w241:bool[])
              n172 = Boolean Array To Number(Boolean array=w241) -> (number=w240:u32)
              n173 = case shown="4, 6" w240 {
                tunnel: [Orca_Data_Spooler_Actions."Exit" ("y") Orca_Data_Spooler_Actions."Copy JSON Files" ("y") Orca_Data_Spooler_Actions."Update Log" ("y")] -> w239
                frame Default {
                }
                frame 2 {
                }
                frame 4, 6 {
                }
              }
            }
            frame "Update Log" {
              n174 = Get Notifier Status(notifier=w281) -> (current notification=w265:T5)  [unwired: 1 in, 4 out]
              n175 = Preview Queue Element(queue=w282) -> (element=w283:path)  [unwired: 2 in, 3 out]
              n176 = Unbundle By Name(w265) -> ("Transfer Log"=w264:path)
              n177 = Strip Path(path=w283) -> (name=w266:string)  [unwired: 1 out]
              n178 = Open/Create/Replace File(file path (use dialog)=w264, operation (0:open)=T16."open or create", access (0:read/write)=enum16{"read/write", "read-only", "write-only"}."read/write") -> (refnum out=w278:refnum<file>, error out=w277:errorcluster)  [unwired: 3 in, 1 out]
              n179 = Bundle By Name(cluster=T17 {"File Name"="", "Status"=""} ("Transfer Log Type"), "File Name"=w266, "Status"="Copying") -> (w267:T17)
              n180 = Read from Text File(file (use dialog)=w278, error in=w277) -> (refnum out=w272:refnum<file>, text=w276:string, error out=w275:errorcluster)  [unwired: 2 in, 1 out]
              n181 = Unflatten From JSON(JSON string=w276, type and defaults=T17[] [], error in (no error)=w275) -> (value=w273:T17[], error out=w274:errorcluster)  [unwired: 4 in]
              n182 = case shown="No Error" w274 {
                tunnel: w273 -> [w295 _]
                tunnel: w272 -> [w287 w301]
                tunnel: w267 -> [w285 w296]
                frame No Error {
                  n183 = Build Array (concatenate)(w295, w285) -> (w294:T17[])
                  n184 = Set File Position(offset (in bytes) (0)=i64 0, refnum=w287, from (0:start)=enum16{"start", "end", "current"}."start") -> (refnum out=w286:refnum<file>)  [unwired: 1 in, 1 out]
                  n185 = Flatten To JSON(anything=w294) -> (JSON string=w293:string, 11:w290:errorcluster)  [unwired: 2 in]
                  n186 = Write to Text File(file (use dialog)=w286, text=w293, error in=w290) -> (refnum out=w292:refnum<file>, error out=w291:errorcluster)  [unwired: 1 in, 1 out]
                  n187 = Close File(refnum=w292, error in=w291) -> ()  [unwired: 2 out]
                }
                frame Error {
                  # "File just created, add first data."
                  n188 = Build Array(w296) -> (w300:T17[])
                  n189 = Flatten To JSON(anything=w300) -> (JSON string=w299:string)  [unwired: 2 in, 1 out]
                  n190 = Write to Text File(file (use dialog)=w301, text=w299) -> (refnum out=w298:refnum<file>, error out=w297:errorcluster)  [unwired: 2 in, 1 out]
                  n191 = Close File(refnum=w298, error in=w297) -> ()  [unwired: 2 out]
                }
              }
            }
            frame "Copy File" {
              n192 = Get Notifier Status(notifier=w315) -> (notifier out=w309:refnum<notifier>, current notification=w314:T5)  [unwired: 1 in, 3 out]
              n193 = Dequeue Element(queue=w316) -> (element=w311:path)  [unwired: 2 in, 3 out]
              n194 = Unbundle By Name(w314) -> ("Transfer Log"=w306:path, "Source"=w304:path, "Destination"=w303:path)
              n195 = Path To String(path=w311) -> (string=→"Current File":string)
              n196 = Strip Path(path=w311) -> (name=w313:string)  [unwired: 1 out]
              n197 = Equal?(x=w304, y=w303) -> (x = y?=w302:bool)
              n198 = Build Path(base path=w303, name or relative path=w313) -> (appended path=w312:path)
              n199 = case shown="False" w302 {
                tunnel: w312 -> [w325 _]
                tunnel: w311 -> [w324 _]
                tunnel: w309 -> [w323 w368]
                tunnel: [w320 w364] -> w308
                tunnel: [w318 TRUE] -> w307
                frame False {
                  # "Copy Result"
                  n200 = dll-call lib="D:/Microscope-Control/Tools/Copy File with Progress/Copy File DLL/x64/Release/Copy File DLL.dll" fn="getPointerU16"("Variable"=u16 0) -> ("Pointer Value"=w330:u64)  [unwired: 4 in, 2 out]
                  n201 = dll-call lib="D:/Microscope-Control/Tools/Copy File with Progress/Copy File DLL/x64/Release/Copy File DLL.dll" fn="getPointerINT"("Variable"=-1) -> ("Pointer Value"=w332:u64)  [unwired: 4 in, 2 out]
                  n202 = Path To String(path=w324) -> (string=w329:string)
                  n203 = Path To String(path=w325) -> (string=w328:string)
                  n204 = dll-call lib="D:/Microscope-Control/Tools/Copy File with Progress/Copy File DLL/x64/Release/Copy File DLL.dll" fn="copyFile"("Source File"=w329, "Destination File"=w328, "Update Value Pointer"=w330, "Copy Result Pointer"=w332) -> ("Success"=w327:i32)  [unwired: 7 in, 2 out]
                  n205 = while {
                    tunnel: w330 -> [w343]
                    tunnel: w332 -> [w342]
                    tunnel: w323 -> [w340]
                    tunnel: [w335] -> w322
                    stop <- w341 stop-if-true
                    n206 = Get Notifier Status(notifier=w340) -> (current notification=w339:T5)  [unwired: 1 in, 4 out]
                    n207 = Unbundle By Name(w339) -> ("Actions"=w338:T4)
                    n208 = Wait (ms)(milliseconds to wait=u32 75) -> ()  [unwired: 1 out]
                    n209 = Equal?(x=Orca_Data_Spooler_Actions."Abort", y=w338) -> (x = y?=w335:bool)
                    n210 = Or(x=w335, y="Skip File") -> (x .or. y?=w336:bool)
                    n211 = case shown="False" w336 {
                      tunnel: w343 -> [w353 w355]
                      tunnel: w342 -> [w352 _]
                      tunnel: [w351 TRUE] -> w341
                      frame False {
                        n212 = dll-call lib="LabVIEW" fn="MoveBlock"("Pointer to Source"=w353, "Destination"=u16 0, "Bytes to Move"=2) -> ("Destination"=w348:u16)  [unwired: 6 in, 2 out]
                        n213 = dll-call lib="LabVIEW" fn="MoveBlock"("Pointer to Source"=w352, "Destination"=0, "Bytes to Move"=4) -> ("Destination"=w345:i32)  [unwired: 6 in, 2 out]
                        n214 = Split Number(x=w348) -> (lo(x)=→"Transfer Amount (%)":u8)  [unwired: 1 out]
                        n215 = Greater Or Equal To 0?(x=w345) -> (x >= 0?=w351:bool)
                      }
                      frame True {
                        n216 = dll-call lib="LabVIEW" fn="MoveBlock"("Pointer to Source"=w355, "Destination"=u16 0, "Bytes to Move"=2) -> ("Pointer to Source"=w357:u64, "Destination"=w361:u16)  [unwired: 5 in, 2 out]
                        n217 = Split Number(x=w361) -> (lo(x)=w360:u8)  [unwired: 1 out]
                        n218 = Join Numbers(hi=u8 1, lo=w360) -> ((hi.lo)=w356:u16)
                        n219 = dll-call lib="LabVIEW" fn="MoveBlock"("Source"=w356, "Destination Pointer"=w357, "Bytes to Move"=2) -> ()  [unwired: 7 in, 2 out]
                      }
                    }
                  }
                  n220 = Greater Than 0?(x=w327) -> (x > 0?=w318:bool)
                  n221 = Select(t=Orca_Data_Spooler_Actions."Copy JSON Files", s=w322, f=Orca_Data_Spooler_Actions."Wait for File" ("y")) -> (s? t:f=w320:T4)
                }
                frame True {
                  # "If source and destination match, no transfer is needed but we still want to update the log file with a \"success\"."
                  n222 = Get Notifier Status(notifier=w368) -> (current notification=w371:T5)  [unwired: 1 in, 4 out]
                  n223 = Unbundle By Name(w371) -> ("Actions"=w370:T4)
                  n224 = Equal?(x=Orca_Data_Spooler_Actions."Abort", y=w370) -> (x = y?=w365:bool)
                  n225 = Select(t=Orca_Data_Spooler_Actions."Copy JSON Files", s=w365, f=Orca_Data_Spooler_Actions."Wait for File" ("y")) -> (s? t:f=w364:T4)
                }
              }
              n226 = call "Orca Data Spooler Update Log Copy Status.vi"("Transfer Log"=w306, "Copy Success"=w307) -> ("Copy Success (Dup)"=→"Copy Success":bool)  [unwired: 12 in, 1 out]
            }
            frame "Copy JSON Files" {
              n227 = Get Notifier Status(notifier=w380) -> (current notification=w379:T5)  [unwired: 1 in, 4 out]
              n228 = Unbundle By Name(w379) -> ("Destination"=w375:path, "Source"=w376:path)
              n229 = List Folder(path=w376, pattern="*.json") -> (filenames=w377:string[], error out=w374:errorcluster)  [unwired: 2 in, 2 out]
              n230 = for {
                tunnel: w377 -> [w392] mode=indexing
                tunnel: w376 -> [w394]
                tunnel: w375 -> [w393]
                shift-right: [w390] -> _
                shift-left: w374 -> [w391]
                n231 = Build Path(base path=w394, name or relative path=w392) -> (appended path=w389:path)
                n232 = Build Path(base path=w393, name or relative path=w392) -> (appended path=w387:path)
                n233 = call <vilib>:"Check if File or Folder Exists.vi"("path"=w389) -> ("file or folder exists?"=w383:bool, "dup path"=w388:path)  [unwired: 8 in, 1 out]
                n234 = call <vilib>:"Check if File or Folder Exists.vi"("path"=w387) -> ("file or folder exists?"=w385:bool, "dup path"=w386:path)  [unwired: 8 in, 1 out]
                n235 = Not(x=w385) -> (.not. x?=w384:bool)
                n236 = And(x=w384, y=w383) -> (x .and. y?=w382:bool)
                n237 = case shown="True" w382 {
                  tunnel: w391 -> [w395 w400]
                  tunnel: [w395 w399] -> w390
                  tunnel: w388 -> [_ w397]
                  tunnel: w386 -> [_ w396]
                  frame False {
                  }
                  frame True {
                    n238 = Copy(8:w400, 9:FALSE ("overwrite (F)"), 10:w396, 11:w397) -> (0:w399:errorcluster)  [unwired: 1 in, 2 out]
                  }
                }
              }
            }
            frame "Log Done" {
              n239 = Get Notifier Status(notifier=w401) -> (current notification=w407:T5)  [unwired: 1 in, 4 out]
              n240 = Unbundle By Name(w407) -> ("Transfer Log"=w406:path)
              n241 = Open/Create/Replace File(file path (use dialog)=w406, operation (0:open)=T16."open", access (0:read/write)=enum16{"read/write", "read-only", "write-only"}."read/write") -> (refnum out=w412:refnum<file>, error out=w411:errorcluster)  [unwired: 3 in, 1 out]
              n242 = Read from Text File(file (use dialog)=w412, error in=w411) -> (refnum out=w402:refnum<file>, text=w410:string, error out=w409:errorcluster)  [unwired: 2 in, 1 out]
              n243 = Unflatten From JSON(JSON string=w410, type and defaults=T17[] [], error in (no error)=w409) -> (value=w404:T17[], error out=w403:errorcluster)  [unwired: 4 in]
              n244 = case shown="No Error" w403 {
                tunnel: w404 -> [w425 _]
                tunnel: w402 -> [w417 _]
                frame No Error {
                  n245 = Array Size(array=w425) -> (size(s)=w428:i32)
                  n246 = disable-structure shown="Enabled" {
                    disable-tunnel: w417 -> [w429 w434]
                    disable-tunnel: [_ w433] -> w416
                    frame Disabled {
                      n247 = Set File Position(offset (in bytes) (0)=i64 0, refnum=w429, from (0:start)=enum16{"start", "end", "current"}."start") -> ()  [unwired: 1 in, 2 out]
                    }
                    frame Enabled {
                      n248 = Set File Size(6:i64 0 ("size (in bytes)"), 7:w434) -> (3:w433:refnum<file>)  [unwired: 1 in, 1 out]
                    }
                  }
                  n249 = Decrement(x=w428) -> (x-1=w424:i32)
                  n250 = Index Array(array=w425, index=w424) -> (element=w427:T17)
                  n251 = Bundle By Name(cluster=w427, "Status"="Done") -> (w423:T17)
                  n252 = Replace Array Subset(array=w425, new element=w423, index=w424) -> (w422:T17[])
                  n253 = Flatten To JSON(anything=w422) -> (JSON string=w421:string, 11:w420:errorcluster)  [unwired: 2 in]
                  n254 = Write to Text File(file (use dialog)=w416, text=w421, error in=w420) -> (refnum out=w419:refnum<file>, error out=w418:errorcluster)  [unwired: 1 in, 1 out]
                  n255 = Close File(refnum=w419, error in=w418) -> ()  [unwired: 2 out]
                }
                frame Error {
                }
              }
            }
            frame "Exit" {
              n256 = Not(x=w442) -> (.not. x?=w441:bool)
              n257 = Get Notifier Status(notifier=w436) -> (notifier out=w439:refnum<notifier>, current notification=w438:T5)  [unwired: 1 in, 3 out]
              n258 = Bundle By Name(cluster=w438, "Running?"=FALSE) -> (w437:T5)
              n259 = Send Notification(notification=w437, notifier=w439) -> ()  [unwired: 1 in, 2 out]
            }
            frame "Quit" {
              n260 = Not(x=w447) -> (.not. x?=w446:bool)
              n261 = Release Notifier(notifier=w443) -> ()  [unwired: 2 in, 3 out]
              n262 = Release Queue(queue=w444) -> ()  [unwired: 2 in, 3 out]
            }
          }
        }
      }
    }
    frame Error {
      n263 = Release Notifier(notifier=w549, error in (no error)=w552) -> (error out=w551:errorcluster)  [unwired: 1 in, 2 out]
      n264 = Release Notifier(notifier=w550, error in (no error)=w551) -> (error out=w547:errorcluster)  [unwired: 1 in, 2 out]
      n265 = Release Notifier(notifier=w548, error in (no error)=w547) -> (error out=→"Start Up Error":errorcluster)  [unwired: 1 in, 2 out]
    }
  }
  n266 = To Word Integer(number=w51) -> (16bit integer=w54:i16)
  n267 = To Word Integer(number=w52) -> (16bit integer=w55:i16)
  n268 = Add(x=w45, y=w48) -> (x+y=w47:i16)
  n269 = Compound Arithmetic op=ADD(w56, w54, w55, i16 12 ("y")) -> (w50:i16)
  n270 = Bundle By Name(cluster=w43, "Right"=w47, "Bottom"=w50) -> (w44:T14)
  n271 = property class="VI"(reference=w42, "Front Panel.PanelBounds"=w44) -> ()  [unwired: 1 in, 2 out]
